vi "DAC Configure.vi"(8 "error in":errorcluster, 11 "DAC RTD Temp in":refnum<class "DAC RTD Temp.lvclass">) -> (0 "error out":errorcluster, 3 "DAC RTD Temp out":refnum<class "DAC RTD Temp.lvclass">)   [LabVIEW 2019, in "DAC.lvlib" / "DAC RTD Temp.lvclass"]
uses:
  DAC RTD Temp.lvclass
  C:/Users/krio/Documents/LV_Projects/test-stand/App/DAC/DAC.lvclass
  DAC.lvclass/DAC.ctl
  DAC RTD Temp.lvclass/DAC RTD Temp.ctl
  <vilib>/DAQmx/create/channels.llb/DAQmx Create Channel (AI-Temperature-RTD).vi
  DAC.lvclass
  <resource>/objmgr/daqmx.rc
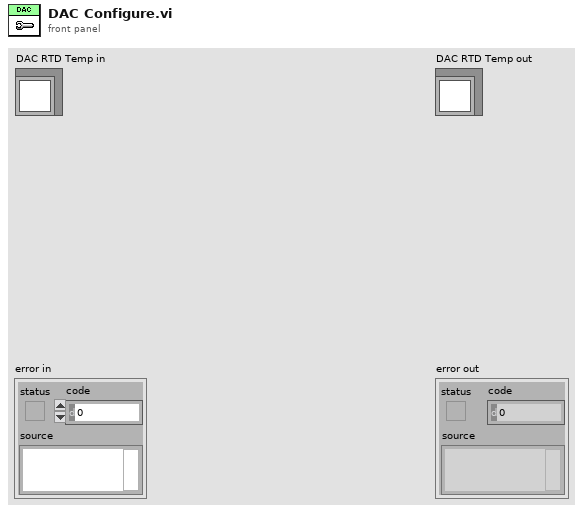
[diagram p1: front panel]
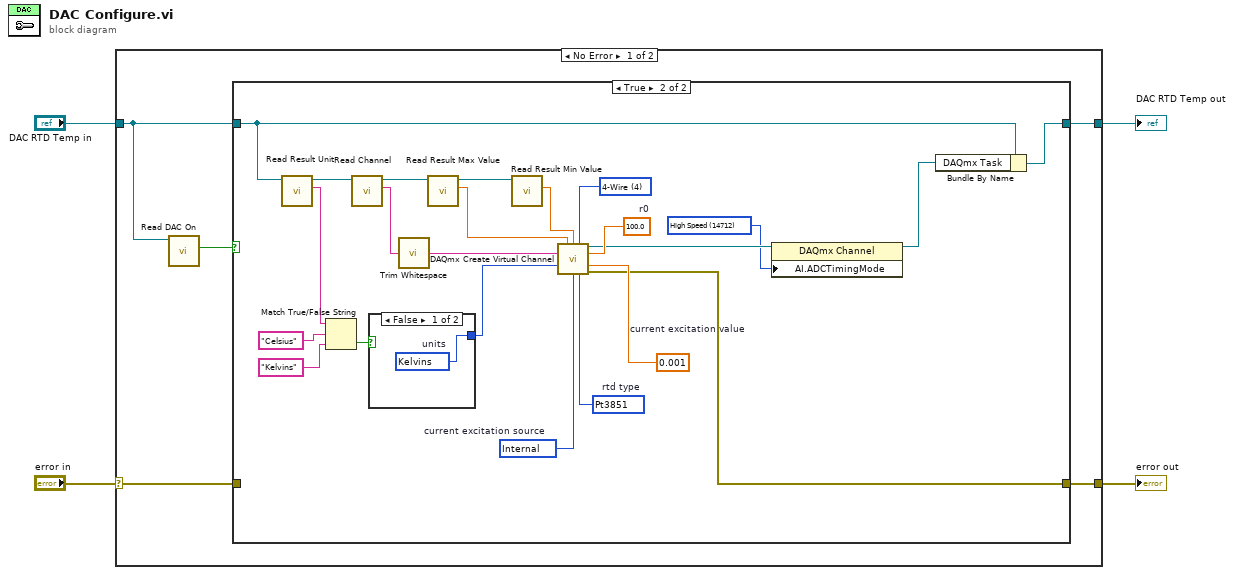
[diagram p0: block diagram]
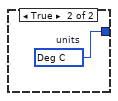
[diagram p3: hidden frame]
diagram:
  n1 = case shown="No Error" "error in" {
    selector: "error in" -> [w6 w38]
    tunnel: [w5 w38] -> w4
    tunnel: [w7 w37] -> w3
    tunnel: "DAC RTD Temp in" -> [w9 w37]
    frame No Error {
      n2 = call "Read DAC On.vi"("DAC in"=w9) -> ("DAC On"=w8:bool)  [unwired: 8 in, 2 out]
      n3 = case shown="True" w8 {
        tunnel: w9 -> [w11 w22]
        tunnel: [w11 w34] -> w7
        tunnel: w6 -> [w10 _]
        tunnel: [w10 w14] -> w5
        frame False {
        }
        frame True {
          w12 = 14712 items=["Automatic"=16097, "High Resolution"=10195, "High Speed"=14712, "Best 50 Hz Rejection"=14713, "Best 60 Hz Rejection"=14714, "Custom"=10137] ("AI.ADCTimingMode")
          w28 = 0.001  # current excitation value
          w29 = 10071 items=["Pt3750"=12481, "Pt3851"=10071, "Pt3911"=12482, "Pt3916"=10069, "Pt3920"=10053, "Pt3928"=12483, "Custom"=10137]  # rtd type
          w30 = 10200 items=["Internal"=10200, "External"=10167, "None"=10230]  # current excitation source
          w31 = 100.0  # r0
          w32 = 4 items=["2-Wire"=2, "3-Wire"=3, "4-Wire"=4] ("resistance configuration")
          n4 = call "Read Result Unit.vi"("DAC in"=w22) -> ("Unit"=w23:string, "DAC out"=w18:refnum<class "DAC RTD Temp.lvclass">)  [unwired: 8 in, 1 out]
          n5 = Match True/False String(2:"Kelvins" ("false string"), 3:"Celsius" ("true string"), 4:w23) -> (0:w24:bool)  [unwired: 1 out]
          n6 = call "Read Channel.vi"("DAC in"=w18) -> ("Channel"=w33:string, "DAC out"=w19:refnum<class "DAC RTD Temp.lvclass">)  [unwired: 8 in, 1 out]
          n7 = case shown="False" w24 {
            tunnel: [w35 w36] -> w21
            frame False {
              w35 = 10325 items=["Deg C"=10143, "Deg F"=10144, "Kelvins"=10325, "Deg R"=10145, "From Custom Scale"=10065]  # units
            }
            frame True {
              w36 = 10143 items=["Deg C"=10143, "Deg F"=10144, "Kelvins"=10325, "Deg R"=10145, "From Custom Scale"=10065]  # units
            }
          }
          n8 = call <vilib>:"Trim Whitespace.vi"("string"=w33) -> ("trimmed string"=w27:string)  [unwired: 1 in]
          n9 = call "Read Result Max Value.vi"("DAC in"=w19) -> ("Max Value"=w17:dbl, "DAC out"=w20:refnum<class "DAC RTD Temp.lvclass">)  [unwired: 8 in, 1 out]
          n10 = call "Read Result Min Value.vi"("DAC in"=w20) -> ("Min Value"=w16:dbl)  [unwired: 8 in, 2 out]
          n11 = call-poly <vilib>:"DAQmx Create Virtual Channel.vi"("maximum value"=w17, "minimum value"=w16, "resistance configuration"=w32, "physical channels"=w27, "r0"=w31, "units"=w21, "current excitation value"=w28, "current excitation source"=w30, "rtd type"=w29) -> ("task out"=w15:refnum<k21>, "error out"=w14:errorcluster)  [unwired: 5 in]
          n12 = property class="DAQmx Channel"(reference=w15, "AI.ADCTimingMode"=w12) -> (reference out=w13:refnum<k21>)  [unwired: 1 in, 1 out]
          n13 = Bundle By Name(cluster=w22, "DAQmx Task"=w13) -> (w34:refnum<class "DAC RTD Temp.lvclass">)
        }
      }
    }
    frame Error {
    }
  }
  "error out" <- w4
  "DAC RTD Temp out" <- w3
